vi "Open Venv Session.vi"(8 "error in":errorcluster, 11 "Venv":path) -> (0 "error out":errorcluster, 3 "session out":refnum<k35>)   [LabVIEW 2026]
doc: "This VI extracts the python version from the provided environment and opens a venv session."
uses:
  <vilib>/Python/Open Venv Python Session.vi
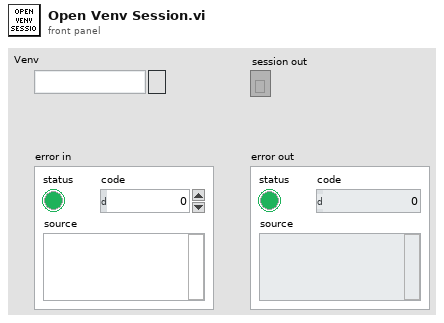
[diagram p1: front panel]
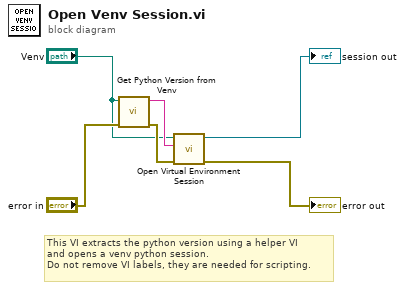
[diagram p0: block diagram]
diagram:
  # "This VI extracts the python version using a helper VI\nand opens a venv python session.\nDo not remove VI labels, they are needed for scripting."
  n1 = call "Get Python Version from Venv.vi"("error in"="error in", "venv"="Venv") -> ("error out"=w6:errorcluster, "Python Version"=w3:string)  [unwired: 8 in]
  n2 = call-poly <vilib>:"Open Virtual Environment Session.vi"("error in (no error)"=w6, "Python version"=w3, "Env path"="Venv") -> ("error out"=→"error out":errorcluster, "session out"=→"session out":refnum<k35>)  [unwired: 7 in]
